vi "Tooling Playground.vi"() -> ()   [LabVIEW 2019]
uses:
  Classes/Settings/Setting Database/Typedefs/PublicEvents--Setting Database.PathsUpdated.ctl
  Classes/Settings/Path Settings/Path Settings.lvclass
  Classes/Settings/Setting Database/Typedefs/PublicEvents--Setting Database.RectanglesUpdated.ctl
  Classes/Settings/Rectangle Settings/Rectangle Settings.lvclass
  C:/Users/Albro/Documents/GitHub/AFM-Lithography/lvsrc/Classes/Settings/ObjectSettings/ObjectSettings.lvclass
  Classes/Settings/Setting Database/Typedefs/PublicEvents--Setting Database.FunnelsUpdated.ctl
  Classes/Settings/Funnel Settings/Funnel Settings.lvclass
  Classes/Settings/Setting Database/Typedefs/PublicEvents--Setting Database.DotsUpdated.ctl
  Classes/Settings/Dot Settings/Dot Settings.lvclass
  Classes/Parse/ParsePaths/Path.lvclass
  Classes/Parse/Rectangle/Rectangle.lvclass
  Classes/Parse/Image/SVGImage.lvclass
  Classes/Parse/Dot/Dot.lvclass
  Classes/Parse/ParsePaths/Path.lvclass/Path.ctl
  Classes/Tool/Tool Data/Tool Data/Tool Data.lvclass
  Classes/Tool/Tool Rectangle/Tool Rectangle.lvclass
  Classes/Settings/ObjectSettings/ObjectSettings.lvclass/ObjectSettings.ctl
  Classes/Settings/Rectangle Settings/Rectangle Settings.lvclass/Rectangle Settings.ctl
  Classes/Parse/Transform/Transform.lvclass/Transform.ctl
  Classes/Tool/Tool Funnel/Tool Funnel.lvclass
  subVIs/typedefs/Schedule Types/Schedule--Formula.ctl
  Classes/Tool/Tool Path/Tool Path.lvclass
  Classes/Settings/Path Settings/Path Settings.lvclass/Path Settings.ctl
  <vilib>/Analysis/baseanly.llb/Real A x B.vi
  Classes/Parse/ParsePaths/Read Transforms.vi
  <userlib>/_OpenG.lib/md5/md5.llb/MD5 Message Digest (Hexadecimal String)__ogtk.vi
  Classes/Parse/PathCommands/Point.ctl
  Classes/Parse/PathCommands/PathCommands.lvclass
  Classes/Parse/Transform/Transform.lvclass
  Classes/Settings/ObjectSettings/ObjectSettings.lvclass
  Classes/Tool/Tool Object/Tool Object.lvclass
  Classes/Parse/PathCommands.Moveto/PathCommands.MoveTo.lvclass
  Classes/Parse/PathCommands.LineTo/PathCommands.LineTo.lvclass
  Classes/Parse/PathCommands.CurveTo/PathCommands.CurveTo.lvclass
  Classes/Parse/PathCommands.ClosePath/PathCommands.ClosePath.lvclass
  Classes/Parse/CSSProperties/CSSProperties.lvclass
  Classes/Parse/Transform.Translate/Transform.Translate.lvclass
  Classes/Parse/Transform.Matrix/Transform.Matrix.lvclass
  Classes/Settings/Setting Database/Setting Database.lvclass
  <vilib>/Analysis/NI_AALBase.lvlib
panel:
  out "GUID":string
  out "Object Sorting":u32
  out "Array":u32[](array[numeric])
  out "Numeric":i32
  out "Rect":u32
  out "Funnel":u32
  out "Path":u32
  in  "Fill Spacing":dbl=2.0 format="%#_13g"
  in  "Fill Orientation":u16(ring) items=["Horizontal", "Vertical"]
  out "XY Graph":cluster{dbl[], dbl[]}[](graph)
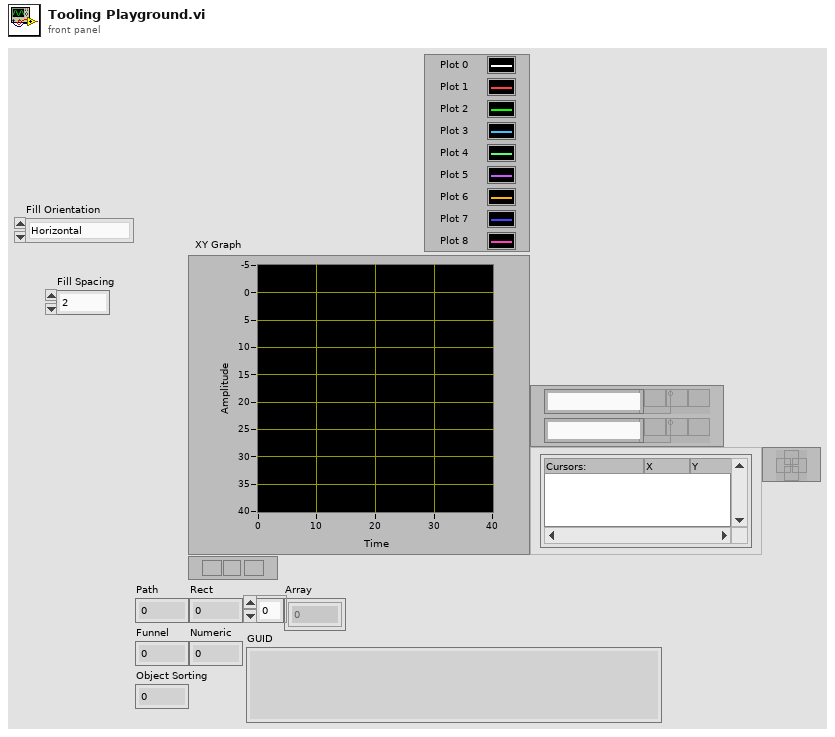
[diagram p1: front panel]
types:
  T1 = cluster{"Paths":refnum<class "Path.lvclass">[], "Rectangles":refnum<class "Rectangle.lvclass">[], "SVGImage":refnum<class "SVGImage.lvclass">, "Dots":refnum<class "Dot.lvclass">[]}
  T2 = typedef "Setting Database.lvclass/PublicEvents--Setting Database.PathsUpdated.ctl" = refnum<class "Path Settings.lvclass">[]
  T3 = typedef "Setting Database.lvclass/PublicEvents--Setting Database.RectanglesUpdated.ctl" = refnum<class "Rectangle Settings.lvclass">[]
  T4 = typedef "Setting Database.lvclass/PublicEvents--Setting Database.FunnelsUpdated.ctl" = refnum<class "Funnel Settings.lvclass">[]
  T5 = typedef "Setting Database.lvclass/PublicEvents--Setting Database.DotsUpdated.ctl" = refnum<class "Dot Settings.lvclass">[]
  T6 = cluster{"Paths":T2, "Rectangles":T3, "Funnels":T4, "Dots":T5}
  T7 = typedef "PathCommands.lvclass/Point.ctl" = cluster{"X":dbl, "Y":dbl}
  T8 = typedef "NI_Matrix.lvlib/RealMatrix.ctl" = dbl[][]
  T9 = typedef "Schedule--Formula.ctl" = cluster{"formula":string, "formula length (nm)":dbl, "formula resolution (nm)":dbl}
  T10 = cluster{"Command Type":string, "Coordinates":cluster{"X":dbl, "Y":dbl}[]}[]
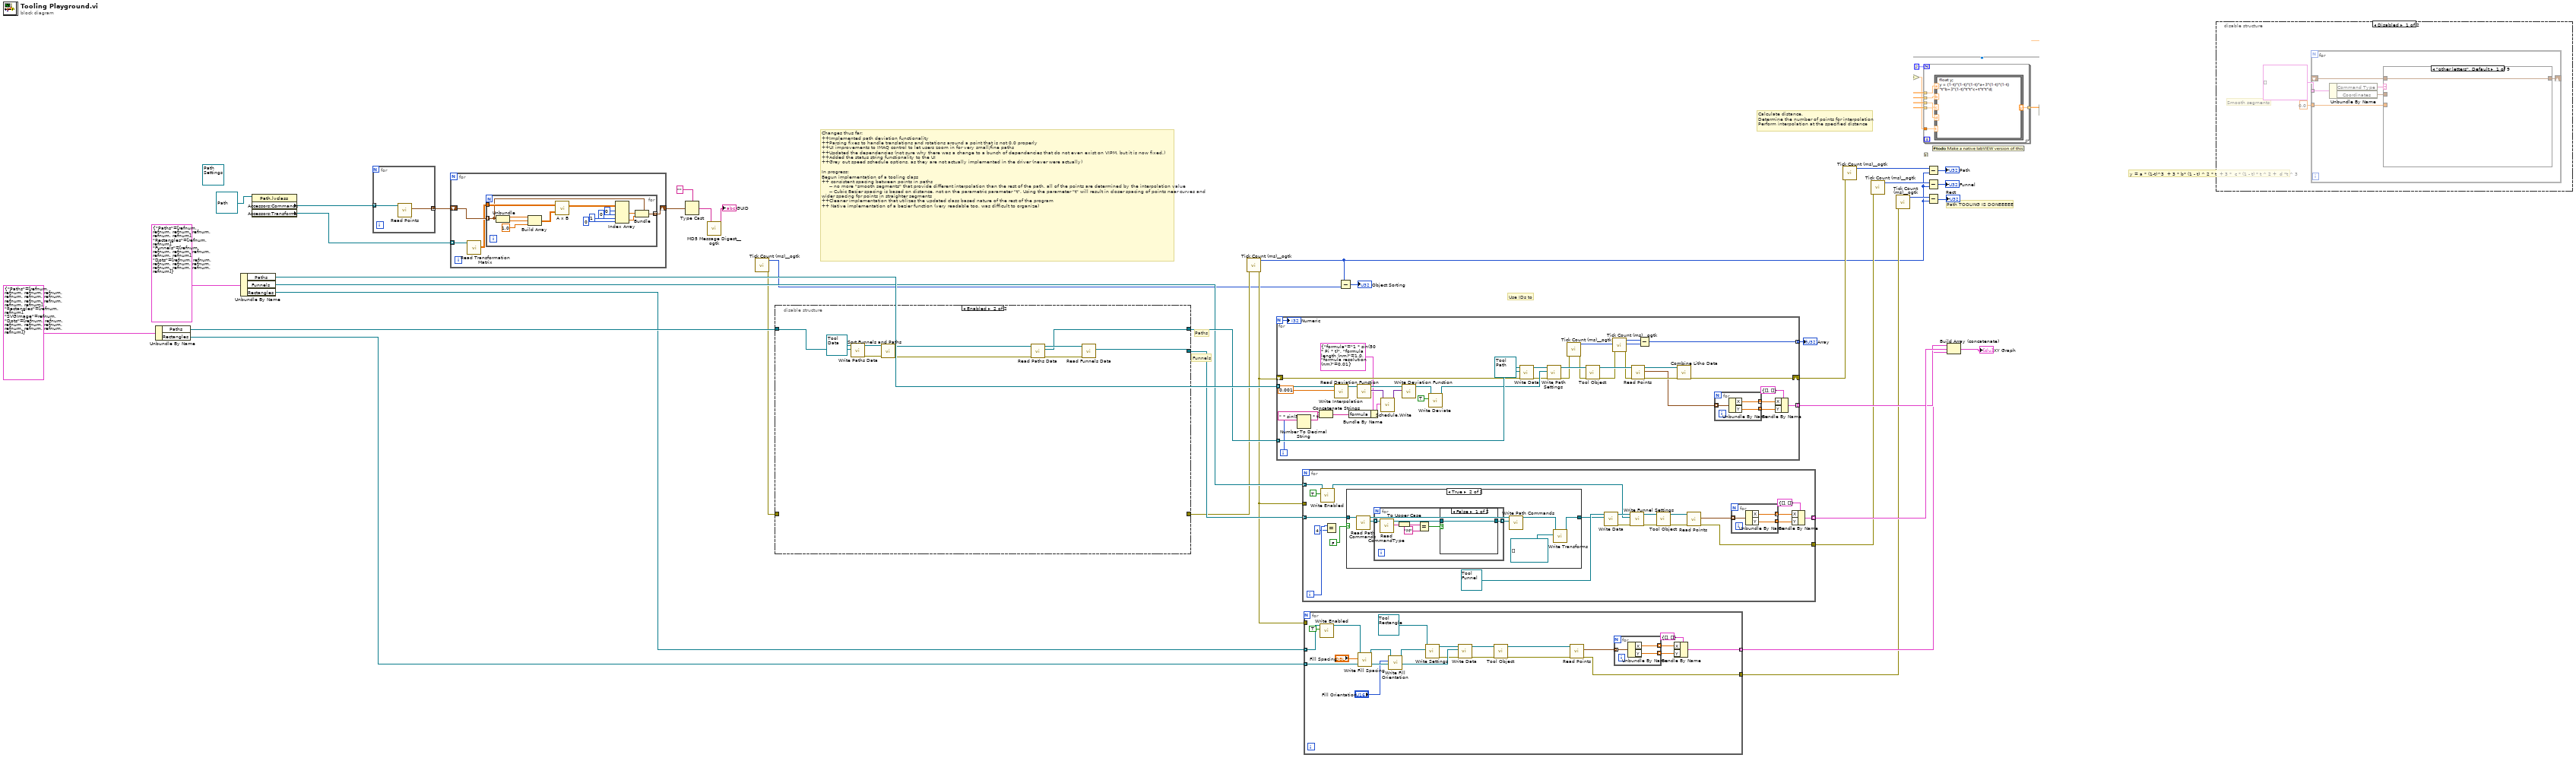
[diagram p0: block diagram]
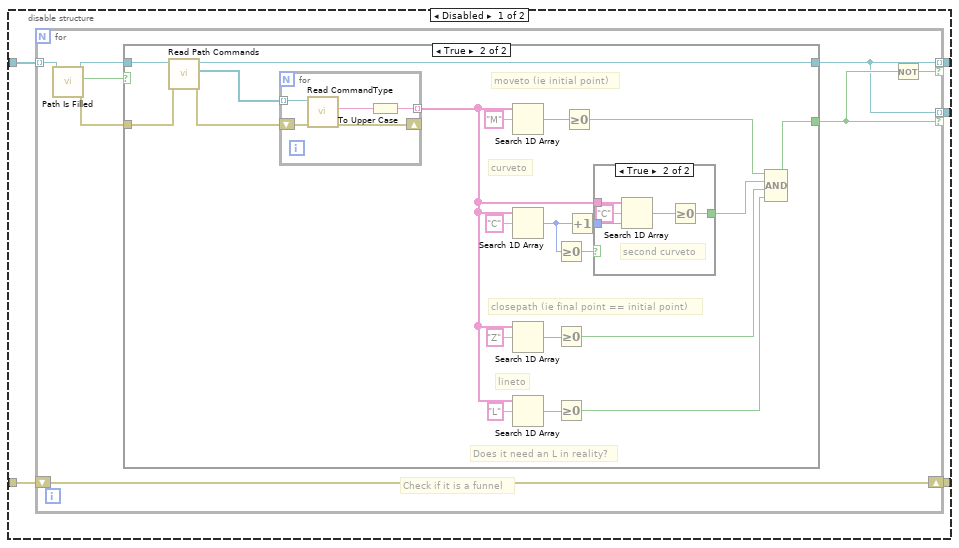
[diagram p2: hidden frame]
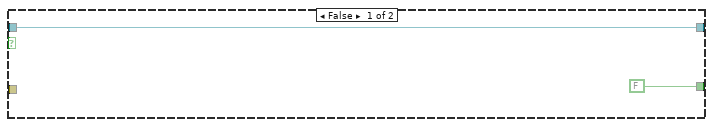
[diagram p3: hidden frame]
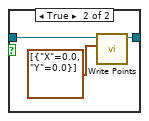
[diagram p6: hidden frame]
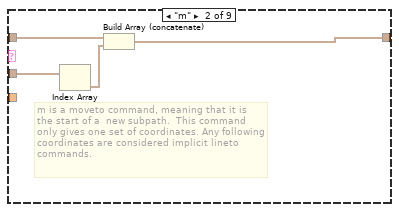
[diagram p7: hidden frame]
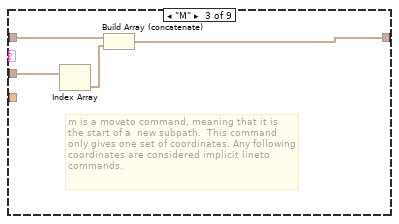
[diagram p8: hidden frame]
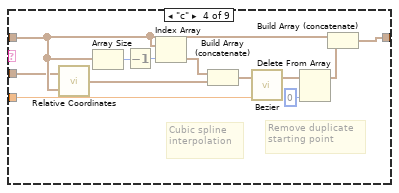
[diagram p9: hidden frame]
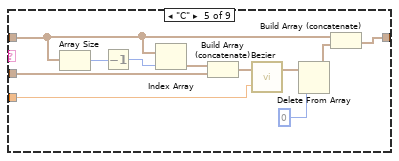
[diagram p10: hidden frame]
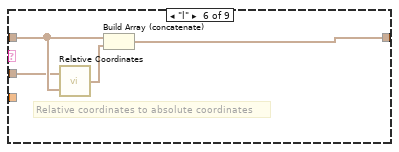
[diagram p11: hidden frame]
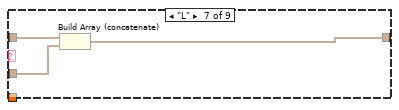
[diagram p12: hidden frame]
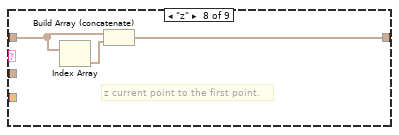
[diagram p13: hidden frame]
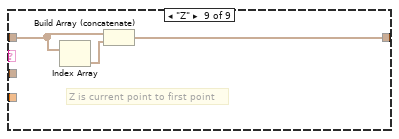
[diagram p14: hidden frame]
diagram:
  (unwired) refnum<class "Path Settings.lvclass"> refnum ("Path Settings.lvclass")
  # "Use IDs to"
  # "Changes thus far:\n++Implemented path deviation functionality\n++Parsing fixes to handle translations and rotations around a point that is not 0,0 properly\n++UI improvements to IMAQ control to let users zoom in for very small/fine paths\n++Updated the dependencies (not sure why there was a change to a bunch of dependencies that do not even exist on VIPM, but it is now fixed.)\n++Added the status string functionality to the UI\n++Grey out speed schedule options, as they are not actually implemented in the driver (never were actually)\n\nIn progress: \nBegun implementation of a tooling class\n++ consistent spacing between points in paths \n     -- no more \"smooth segments\" that provide different interpolation than the rest of the path, all of the points are determined by the interpolation value\n     -- Cubic Bezier spacing is based on distance, not on the parametric parameter \"t\". Using the parameter \"t\" will result in closer spacing of points near curves and wider spacing for points in straighter segments\n++Cleaner implementation that utilizes the updated class based nature of the rest of the program\n++ Native implementation of a bezier function (very readable too, was difficult to organize)"
  # "Path TOOLING IS DONEEEEE"
  # "Calculate distance.\nDetermine the number of points for interpolation\nPerform interpolation at the specified distance"
  # "y = a * (1-t)^3  + 3 * b* (1 - t) ^ 2 * t  + 3 *  c * (1 - t) * t ^ 2 +  d *t ^ 3"
  # "Funnels"
  # "Paths"
  n1 = Unbundle By Name(T1 {"Paths"=[refnum, refnum, refnum, refnum, refnum, refnum, refnum, refnum, refnum, refnum, refnum, refnum], "Rectangles"=[refnum, refnum], "SVGImage"=refnum, "Dots"=[refnum, refnum, refnum, refnum, refnum, refnum, refnum, refnum, refnum]}) -> ("Paths"=w37:refnum<class "Path.lvclass">[], "Rectangles"=w29:refnum<class "Rectangle.lvclass">[])
  n2 = Unbundle By Name(T6 {"Paths"=[refnum, refnum, refnum, refnum, refnum, refnum], "Rectangles"=[refnum, refnum], "Funnels"=[refnum, refnum, refnum, refnum, refnum, refnum], "Dots"=[refnum, refnum, refnum, refnum, refnum, refnum, refnum, refnum, refnum]} ("Response")) -> ("Paths"=w36:T2, "Funnels"=w33:T4, "Rectangles"=w28:T3)
  n3 = property class="Path.lvclass"(reference=refnum<class "Path.lvclass"> refnum ("Path.lvclass")) -> ("Accessors:Commands"=w7:refnum<class "PathCommands.lvclass">[], "Accessors:Transforms"=w6:refnum<class "Transform.lvclass">[])  [unwired: 1 in, 2 out]
  n4 = for {
    tunnel: w7 -> [w39] mode=indexing
    tunnel: [w38] -> w5 mode=concatenating
    n5 = call-dynamic "Read Points.vi"("PathCommands in"=w39) -> ("Points"=w38:T7[])  [unwired: 8 in, 2 out]
  }
  n6 = for {
    tunnel: w6 -> [w43] mode=indexing
    shift-right: [w40] -> w4
    shift-left: w5 -> [w42]
    n7 = call "Read Transformation Matrix.vi"("Transform in"=w43) -> ("Real Matrix"=w41:T8)  [unwired: 8 in, 2 out]
    n8 = for {
      tunnel: w41 -> [w55]
      tunnel: w42 -> [w48] mode=indexing
      tunnel: [w47] -> w40 mode=indexing
      n9 = Unbundle(w48) -> ("X"=w57:dbl, "Y"=w56:dbl)
      n10 = Build Array(w57, w56, 1.0) -> (w44:T8)
      n11 = call-poly <vilib>:"A x B.vi"("B"=w44, "A"=w55) -> ("A x B"=w54:T8)  [unwired: 1 out]
      n12 = Index Array(array=w54, index (row) #1=0 ("index (row)"), index (col) #1=0 ("index (col)"), index (row) #2=1 ("index (row)"), index (col) #2=0 ("index (col)")) -> (element #1=w50:dbl, element #2=w49:dbl)
      n13 = Bundle(cluster=w48, "X"=w50, "Y"=w49) -> (w47:T7)
    }
  }
  n14 = Type Cast(type="", x=w4) -> (*(type *) &x=w2:string)
  n15 = call-poly <userlib>:"MD5 Message Digest__ogtk.vi"("Message"=w2) -> ("MD5 Message Digest"=→"GUID":string)
  n16 = call <userlib>:"Tick Count (ms)__ogtk.vi"() -> ("error out"=w12:errorcluster, "millisecond timer value"=w10:u32)  [unwired: 10 in]
  n17 = disable-structure shown="Enabled" {
    disable-tunnel: w37 -> [w62 w114]
    disable-tunnel: [w61 w108] -> w35
    disable-tunnel: [w60 w107] -> w34
    disable-tunnel: [w59 _] -> w13
    disable-tunnel: w12 -> [w58 _]
    frame Disabled {
      n18 = for {
        tunnel: w62 -> [w64] mode=indexing
        tunnel: [w68] -> w61 mode=indexing if=w70
        tunnel: [w68] -> w60 mode=indexing if=w69
        shift-right: [w66] -> w59
        shift-left: w58 -> [w66]
        # "Check if it is a funnel"
        n19 = call "Path Is Filled.vi"("Path in"=w64) -> ("error out"=w63:errorcluster, "x != y?"=w67:bool, "Path out"=w65:refnum<class "Path.lvclass">)  [unwired: 8 in]
        n20 = case shown="True" w67 {
          tunnel: [FALSE w78] -> w69
          tunnel: w65 -> [w72 w77]
          tunnel: [w72 w76] -> w68
          tunnel: w63 -> [_ w73]
          frame False {
          }
          frame True {
            # "Does it need an L in reality?"
            # "lineto"
            # "closepath (ie final point == initial point)"
            # "curveto"
            # "moveto (ie initial point)"
            n21 = call "Read Path Commands.vi"("error in (no error)"=w73, "Path in"=w77) -> ("error out"=w74:errorcluster, "Path Commands"=w75:refnum<class "PathCommands.lvclass">[], "Path out"=w76:refnum<class "Path.lvclass">)  [unwired: 7 in]
            n22 = for {
              tunnel: w75 -> [w104] mode=indexing
              tunnel: [w102] -> w79 mode=indexing
              shift-right: [w100] -> _
              shift-left: w74 -> [w101]
              n23 = call-dynamic "Read CommandType.vi"("error in (no error)"=w101, "PathCommands in"=w104) -> ("error out"=w100:errorcluster, "CommandType"=w103:string)  [unwired: 7 in, 1 out]
              n24 = To Upper Case(1:w103) -> (0:w102:string)
            }
            n25 = Search 1D Array(1D array=w79, element="M") -> (index of element=w91:i32)  [unwired: 1 in]
            n26 = Search 1D Array(1D array=w79, element="C") -> (index of element=w90:i32)  [unwired: 1 in]
            n27 = Search 1D Array(1D array=w79, element="Z") -> (index of element=w87:i32)  [unwired: 1 in]
            n28 = Search 1D Array(1D array=w79, element="L") -> (index of element=w82:i32)  [unwired: 1 in]
            n29 = Greater Or Equal To 0?(x=w90) -> (x >= 0?=w89:bool)
            n30 = Greater Or Equal To 0?(x=w87) -> (x >= 0?=w84:bool)
            n31 = Greater Or Equal To 0?(x=w82) -> (x >= 0?=w80:bool)
            n32 = Greater Or Equal To 0?(x=w91) -> (x >= 0?=w86:bool)
            n33 = Increment(x=w90) -> (x+1=w83:i32)
            n34 = case shown="True" w89 {
              selector: w89 -> [w94 _]
              tunnel: w83 -> [_ w99]
              tunnel: w79 -> [_ w98]
              tunnel: [w94 w96] -> w85
              frame False {
              }
              frame True {
                # "second curveto"
                n35 = Search 1D Array(1D array=w98, element="C", start index (0)=w99) -> (index of element=w97:i32)
                n36 = Greater Or Equal To 0?(x=w97) -> (x >= 0?=w96:bool)
              }
            }
            n37 = Compound Arithmetic op=AND(w86, w85, w84, w80) -> (w78:bool)
          }
        }
        n38 = Not(x=w69) -> (.not. x?=w70:bool)
      }
    }
    frame Enabled {
      n39 = call-dynamic "Write Paths Data.vi"("Paths"=w114, "Tool Data in"=refnum<class "Tool Data.lvclass"> refnum) -> ("error out"=w111:errorcluster, "Tool Data out"=w112:refnum<class "Tool Data.lvclass">)  [unwired: 8 in]
      n40 = call "Sort Funnels and Paths.vi"("error in (no error)"=w111, "Tool Data in"=w112) -> ("error out"=w105:errorcluster, "Tool Data out"=w110:refnum<class "Tool Data.lvclass">)  [unwired: 8 in]
      n41 = call-dynamic "Read Paths Data.vi"("error in (no error)"=w105, "Tool Data in"=w110) -> ("error out"=w106:errorcluster, "Paths"=w108:refnum<class "Path.lvclass">[], "Tool Data out"=w109:refnum<class "Tool Data.lvclass">)  [unwired: 7 in]
      n42 = call-dynamic "Read Funnels Data.vi"("error in (no error)"=w106, "Tool Data in"=w109) -> ("Funnels"=w107:refnum<class "Path.lvclass">[])  [unwired: 7 in, 2 out]
    }
  }
  n43 = call <userlib>:"Tick Count (ms)__ogtk.vi"("error in (no error)"=w13) -> ("error out"=w24:errorcluster, "millisecond timer value"=w11:u32)  [unwired: 9 in]
  n44 = for {
    N -> [w128]
    tunnel: w36 -> [w150] mode=indexing
    tunnel: w35 -> [w152] mode=indexing
    shift-right: [w130] -> w23
    shift-left: w24 -> [w151]
    tunnel: [w132] -> w30 mode=indexing
    tunnel: [w121] -> w14 mode=indexing
    i -> [w118]
    n45 = Number To Decimal String(number=w118) -> (decimal integer string=w117:string)  [unwired: 1 in]
    n46 = Concatenate Strings(w117, " * sin(50 * Pi * t)" ("string")) -> (w115:string)
    n47 = call "Write Interpolation.vi"("Interpolation"=0.001, "Path Settings in"=w150) -> ("Path Settings out"=w145:refnum<class "Path Settings.lvclass">)  [unwired: 8 in, 1 out]
    n48 = Bundle By Name(cluster=T9 {"formula"="1 * sin(50 * Pi * t)", "formula length (nm)"=1.0, "formula resolution (nm)"=0.01} ("Formula"), "formula"=w115) -> (w119:T9)
    n49 = call-dynamic "Read Deviation Function.vi"("Path Settings in"=w145) -> ("Deviation Function"=w147:variant, "Path Settings out"=w148:refnum<class "Path Settings.lvclass">)  [unwired: 8 in, 1 out]
    n50 = call "Schedule.Write.vi"("Data to Write"=w119, "LUT In"=w147) -> ("LUT Out"=w146:variant)  [unwired: 8 in, 1 out]
    n51 = call-dynamic "Write Deviation Function.vi"("Deviation Function"=w146, "Path Settings in"=w148) -> ("Path Settings out"=w144:refnum<class "Path Settings.lvclass">)  [unwired: 8 in, 1 out]
    n52 = call-dynamic "Write Deviate.vi"("Deviate"=TRUE, "Path Settings in"=w144) -> ("Path Settings out"=w143:refnum<class "Path Settings.lvclass">)  [unwired: 8 in, 1 out]
    n53 = call-dynamic "Write Data.vi"("error in (no error)"=w151, "Path.lvclass"=w152, "Tool Path in"=refnum<class "Tool Path.lvclass"> refnum) -> ("error out"=w140:errorcluster, "Tool Path out"=w141:refnum<class "Tool Path.lvclass">)  [unwired: 7 in]
    n54 = call-dynamic "Write Path Settings.vi"("error in (no error)"=w140, "Path Settings.lvclass"=w143, "Tool Path in"=w141) -> ("error out"=w127:errorcluster, "Tool Path out"=w139:refnum<class "Tool Path.lvclass">)  [unwired: 7 in]
    n55 = call <userlib>:"Tick Count (ms)__ogtk.vi"("error in (no error)"=w127) -> ("error out"=w126:errorcluster, "millisecond timer value"=w122:u32)  [unwired: 9 in]
    n56 = call-dynamic "Tool Object.vi"("error in (no error)"=w126, "Tool Path in"=w139) -> ("error out"=w125:errorcluster, "Tool Path out"=w138:refnum<class "Tool Path.lvclass">)  [unwired: 8 in]
    n57 = call <userlib>:"Tick Count (ms)__ogtk.vi"("error in (no error)"=w125) -> ("error out"=w124:errorcluster, "millisecond timer value"=w123:u32)  [unwired: 9 in]
    n58 = call-dynamic "Read Points.vi"("error in (no error)"=w124, "Tool Object in"=w138) -> ("error out"=w136:errorcluster, "Points"=w131:T7[], "Tool Object out"=w137:refnum<class "Tool Path.lvclass">)  [unwired: 7 in]
    n59 = Subtract(x=w123, y=w122) -> (x-y=w121:u32)
    n60 = call-dynamic "Combine Litho Data.vi"("error in (no error)"=w136, "Tool Object in"=w137) -> ("error out"=w130:errorcluster)  [unwired: 7 in, 2 out]
    n61 = for {
      tunnel: w131 -> [w155] mode=indexing
      tunnel: [w154] -> w135 mode=indexing
      tunnel: [w153] -> w134 mode=indexing
      n62 = Unbundle By Name(w155) -> ("X"=w154:dbl, "Y"=w153:dbl)
    }
    n63 = Bundle By Name(cluster=cluster{"X":dbl[], "Y":dbl[]} {"X"=[], "Y"=[]} ("input cluster"), "X"=w135, "Y"=w134) -> (w132:cluster{"X":dbl[], "Y":dbl[]})
    "Numeric" <- w128
  }
  "Array" <- w14
  n64 = for {
    tunnel: w34 -> [w168] mode=indexing
    tunnel: w33 -> [w163] mode=indexing
    tunnel: [w157] -> w32 mode=indexing
    tunnel: w24 -> [_]
    tunnel: [w156] -> w22
    i -> [w167]
    n65 = call "Write Enabled.vi"("Enabled"=TRUE, "ObjectSettings in"=w163) -> ("ObjectSettings out"=w164:refnum<class "Funnel Settings.lvclass">)  [unwired: 8 in, 1 out]
    n66 = Equal?(x=w167, y=4) -> ()  [unwired: 1 out]
    n67 = case shown="True" FALSE {
      tunnel: [w180 w182] -> w169
      tunnel: w168 -> [w180 w187]
      frame False {
      }
      frame True {
        n68 = call "Read Path Commands.vi"("Path in"=w187) -> ("Path Commands"=w186:refnum<class "PathCommands.lvclass">[], "Path out"=w185:refnum<class "Path.lvclass">)  [unwired: 8 in, 1 out]
        n69 = for {
          tunnel: w186 -> [w194] mode=indexing
          tunnel: [w188] -> w184 mode=indexing
          n70 = call-dynamic "Read CommandType.vi"("PathCommands in"=w194) -> ("CommandType"=w193:string, "PathCommands out"=w189:refnum<class "PathCommands.lvclass">)  [unwired: 8 in, 1 out]
          n71 = To Upper Case(1:w193) -> (0:w192:string)
          n72 = Equal?(x=w192, y="M") -> (x = y?=w190:bool)
          n73 = case shown="False" w190 {
            tunnel: w189 -> [w195 w198]
            tunnel: [w195 w196] -> w188
            frame False {
            }
            frame True {
              n74 = call-dynamic "Write Points.vi"("Points"=T7[] [{"X"=0.0, "Y"=0.0}], "PathCommands in"=w198) -> ("PathCommands out"=w196:refnum<class "PathCommands.lvclass">)  [unwired: 8 in, 1 out]
            }
          }
        }
        n75 = call "Write Path Commands.vi"("Path Commands"=w184, "Path in"=w185) -> ("Path out"=w183:refnum<class "Path.lvclass">)  [unwired: 8 in, 1 out]
        n76 = call "Write Transforms.vi"("Transforms"=refnum<class "Transform.lvclass">[] [], "Path in"=w183) -> ("Path out"=w182:refnum<class "Path.lvclass">)  [unwired: 8 in, 1 out]
      }
    }
    n77 = call-dynamic "Write Data.vi"("Path.lvclass"=w169, "Tool Path in"=refnum<class "Tool Funnel.lvclass"> refnum ("Tool Funnel in")) -> ("error out"=w174:errorcluster, "Tool Path out"=w175:refnum<class "Tool Funnel.lvclass">)  [unwired: 8 in]
    n78 = call-dynamic "Write Funnel Settings.vi"("error in (no error)"=w174, "Funnel Settings.lvclass"=w164, "Tool Funnel in"=w175) -> ("error out"=w172:errorcluster, "Tool Funnel out"=w173:refnum<class "Tool Funnel.lvclass">)  [unwired: 7 in]
    n79 = call-dynamic "Tool Object.vi"("error in (no error)"=w172, "Tool Funnel in"=w173) -> ("error out"=w170:errorcluster, "Tool Funnel out"=w171:refnum<class "Tool Funnel.lvclass">)  [unwired: 8 in]
    n80 = call-dynamic "Read Points.vi"("error in (no error)"=w170, "Tool Object in"=w171) -> ("error out"=w156:errorcluster, "Points"=w161:T7[])  [unwired: 7 in, 1 out]
    n81 = for {
      tunnel: w161 -> [w179] mode=indexing
      tunnel: [w178] -> w160 mode=indexing
      tunnel: [w177] -> w159 mode=indexing
      n82 = Unbundle By Name(w179) -> ("X"=w178:dbl, "Y"=w177:dbl)
    }
    n83 = Bundle By Name(cluster=cluster{"X":dbl[], "Y":dbl[]} {"X"=[], "Y"=[]} ("input cluster"), "X"=w160, "Y"=w159) -> (w157:cluster{"X":dbl[], "Y":dbl[]})
  }
  n84 = for {
    tunnel: w29 -> [w217] mode=indexing
    tunnel: w28 -> [w212] mode=indexing
    tunnel: [w201] -> w27 mode=indexing
    tunnel: w24 -> [_]
    tunnel: [w199] -> w21
    n85 = call "Write Enabled.vi"("Enabled"=TRUE, "ObjectSettings in"=w212) -> ("ObjectSettings out"=w210:refnum<class "Rectangle Settings.lvclass">)  [unwired: 8 in, 1 out]
    n86 = call "Write Fill Spacing.vi"("Fill Spacing"="Fill Spacing", "Rectangle Settings in"=w210) -> ("Rectangle Settings out"=w208:refnum<class "Rectangle Settings.lvclass">)  [unwired: 8 in, 1 out]
    n87 = call "Write Fill Orientation.vi"("Fill Orientation"="Fill Orientation", "Rectangle Settings in"=w208) -> ("Rectangle Settings out"=w207:refnum<class "Rectangle Settings.lvclass">)  [unwired: 8 in, 1 out]
    n88 = call-dynamic "Write Settings.vi"("Rectangle Settings.lvclass"=w207, "Tool Rectangle in"=refnum<class "Tool Rectangle.lvclass"> refnum) -> ("error out"=w216:errorcluster, "Tool Rectangle out"=w218:refnum<class "Tool Rectangle.lvclass">)  [unwired: 8 in]
    n89 = call-dynamic "Write Data.vi"("error in (no error)"=w216, "Rectangle.lvclass"=w217, "Tool Rectangle in"=w218) -> ("error out"=w214:errorcluster, "Tool Rectangle out"=w215:refnum<class "Tool Rectangle.lvclass">)  [unwired: 7 in]
    n90 = call-dynamic "Tool Object.vi"("error in (no error)"=w214, "Tool Rectangle in"=w215) -> ("error out"=w200:errorcluster, "Tool Rectangle out"=w211:refnum<class "Tool Rectangle.lvclass">)  [unwired: 8 in]
    n91 = call-dynamic "Read Points.vi"("error in (no error)"=w200, "Tool Object in"=w211) -> ("error out"=w199:errorcluster, "Points"=w202:T7[])  [unwired: 7 in, 1 out]
    n92 = for {
      tunnel: w202 -> [w222] mode=indexing
      tunnel: [w221] -> w205 mode=indexing
      tunnel: [w220] -> w204 mode=indexing
      n93 = Unbundle By Name(w222) -> ("X"=w221:dbl, "Y"=w220:dbl)
    }
    n94 = Bundle By Name(cluster=cluster{"X":dbl[], "Y":dbl[]} {"X"=[], "Y"=[]} ("input cluster"), "X"=w205, "Y"=w204) -> (w201:cluster{"X":dbl[], "Y":dbl[]})
  }
  n95 = Subtract(x=w11, y=w10) -> (x-y=→"Object Sorting":u32)
  n96 = call <userlib>:"Tick Count (ms)__ogtk.vi"("error in (no error)"=w23) -> ("millisecond timer value"=w20:u32)  [unwired: 9 in, 1 out]
  n97 = call <userlib>:"Tick Count (ms)__ogtk.vi"("error in (no error)"=w22) -> ("millisecond timer value"=w19:u32)  [unwired: 9 in, 1 out]
  n98 = call <userlib>:"Tick Count (ms)__ogtk.vi"("error in (no error)"=w21) -> ("millisecond timer value"=w18:u32)  [unwired: 9 in, 1 out]
  n99 = Subtract(x=w20, y=w11) -> (x-y=→"Path":u32)
  n100 = Subtract(x=w19, y=w11) -> (x-y=→"Funnel":u32)
  n101 = Subtract(x=w18, y=w11) -> (x-y=→"Rect":u32)
  n102 = Build Array (concatenate)(w30, w32, w27) -> (→"XY Graph":cluster{"X":dbl[], "Y":dbl[]}[])
  n103 = disable-structure shown="Disabled" {
    frame Disabled {
      # "Smooth segments"
      n104 = for {
        tunnel: T10 [] ("Commands") -> [w230] mode=indexing
        shift-right: [w226] -> _
        shift-left: _ -> [w227]
        tunnel: 0.0 ("Smooth Segments") -> [w225]
        n105 = Unbundle By Name(w230) -> ("Command Type"=w229:string, "Coordinates"=w228:cluster{"X":dbl, "Y":dbl}[])
        n106 = case shown="\"other letters\", Default" w229 {
          tunnel: w228 -> [_ w235 w237 w244 w255 w263 w267 _ _]
          tunnel: w227 -> [w231 w234 w238 w250 w261 w265 w269 w271 w275]
          tunnel: [w231 w232 w236 w251 w262 w264 w268 w270 w273] -> w226
          tunnel: w225 -> [_ _ _ w243 w256 _ _ _ _]
          frame "other letters", Default {
          }
          frame "m" {
            # "m is a moveto command, meaning that it is the start of a  new subpath.  This command only gives one set of coordinates. Any following coordinates are considered implicit lineto commands."
            n107 = Index Array(array=w235) -> (element=w233:cluster{"X":dbl, "Y":dbl})  [unwired: 1 in]
            n108 = Build Array (concatenate)(w234, w233) -> (w232:cluster{"X":dbl, "Y":dbl}[])
          }
          frame "M" {
            # "m is a moveto command, meaning that it is the start of a  new subpath.  This command only gives one set of coordinates. Any following coordinates are considered implicit lineto commands."
            n109 = Index Array(array=w237) -> (element=w239:cluster{"X":dbl, "Y":dbl})  [unwired: 1 in]
            n110 = Build Array (concatenate)(w238, w239) -> (w236:cluster{"X":dbl, "Y":dbl}[])
          }
          frame "c" {
            # "Remove duplicate starting point"
            # "Cubic spline interpolation"
            n111 = call "Relative Coordinates.vi"("All Coordinates"=w250, "Command Coordinates"=w244) -> ("Adjusted Command Coordinates"=w248:cluster{"X":dbl, "Y":dbl}[])
            n112 = Array Size(array=w250) -> (size(s)=w246:i32)
            n113 = Decrement(x=w246) -> (x-1=w245:i32)
            n114 = Index Array(array=w250, index=w245) -> (element=w249:cluster{"X":dbl, "Y":dbl})
            n115 = Build Array (concatenate)(w249, w248) -> (w247:cluster{"X":dbl, "Y":dbl}[])
            n116 = call "Bezier.vi"("Segments"=w243, "Parameters"=w247) -> ("Coordinate Array"=w242:cluster{"X":dbl, "Y":dbl}[])  [unwired: 1 out]
            n117 = Delete From Array(array=w242, index=0) -> (array with subset deleted=w241:cluster{"X":dbl, "Y":dbl}[])  [unwired: 1 in, 1 out]
            n118 = Build Array (concatenate)(w250, w241) -> (w251:cluster{"X":dbl, "Y":dbl}[])
          }
          frame "C" {
            n119 = Array Size(array=w261) -> (size(s)=w258:i32)
            n120 = Decrement(x=w258) -> (x-1=w257:i32)
            n121 = Index Array(array=w261, index=w257) -> (element=w260:cluster{"X":dbl, "Y":dbl})
            n122 = Build Array (concatenate)(w260, w255) -> (w259:cluster{"X":dbl, "Y":dbl}[])
            n123 = call "Bezier.vi"("Segments"=w256, "Parameters"=w259) -> ("Coordinate Array"=w254:cluster{"X":dbl, "Y":dbl}[])  [unwired: 1 out]
            n124 = Delete From Array(array=w254, index=0) -> (array with subset deleted=w253:cluster{"X":dbl, "Y":dbl}[])  [unwired: 1 in, 1 out]
            n125 = Build Array (concatenate)(w261, w253) -> (w262:cluster{"X":dbl, "Y":dbl}[])
          }
          frame "l" {
            # "Relative coordinates to absolute coordinates"
            n126 = call "Relative Coordinates.vi"("All Coordinates"=w265, "Command Coordinates"=w263) -> ("Adjusted Command Coordinates"=w266:cluster{"X":dbl, "Y":dbl}[])
            n127 = Build Array (concatenate)(w265, w266) -> (w264:cluster{"X":dbl, "Y":dbl}[])
          }
          frame "L" {
            n128 = Build Array (concatenate)(w269, w267) -> (w268:cluster{"X":dbl, "Y":dbl}[])
          }
          frame "z" {
            # "z current point to the first point."
            n129 = Index Array(array=w271) -> (element=w272:cluster{"X":dbl, "Y":dbl})  [unwired: 1 in]
            n130 = Build Array (concatenate)(w271, w272) -> (w270:cluster{"X":dbl, "Y":dbl}[])
          }
          frame "Z" {
            # "Z is current point to first point"
            n131 = Index Array(array=w275) -> (element=w274:cluster{"X":dbl, "Y":dbl})  [unwired: 1 in]
            n132 = Build Array (concatenate)(w275, w274) -> (w273:cluster{"X":dbl, "Y":dbl}[])
          }
        }
      }
    }
    frame Enabled {
    }
  }
